vi "Broadcast number of frames and run ID.vi"(8 "error in":errorcluster, 10 "CaptureDetectionLoopDataIn":T1={"Period"=-1, "Reset"=FALSE, "Iteration"=0, "Capture"=path "", "Mode"={"Replay"=enum."None", "Record"=enum."None"}, "Replay Run ID"="", "Frame Number"=0, "Core Module ID"=0, "EventRecorderLaunched"=FALSE, "Frame 0 relative seconds"=0.0} {"Frame 0 relative seconds" format="%_19f"}, 11 "Number of frames":u32) -> (0 "error out":errorcluster)   [LabVIEW 2026, in "Launcher.lvlib"]
doc: "_____\nCreated using DQMH Framework: Event Scripter 7.1.2.1547."
uses:
  Launcher.lvlib
  Capture detection loop data--cluster.ctl
  Mode.ctl
  ReplayMode.ctl
  RecordMode.ctl
  Broadcast number of frames and run ID Argument--cluster.ctl
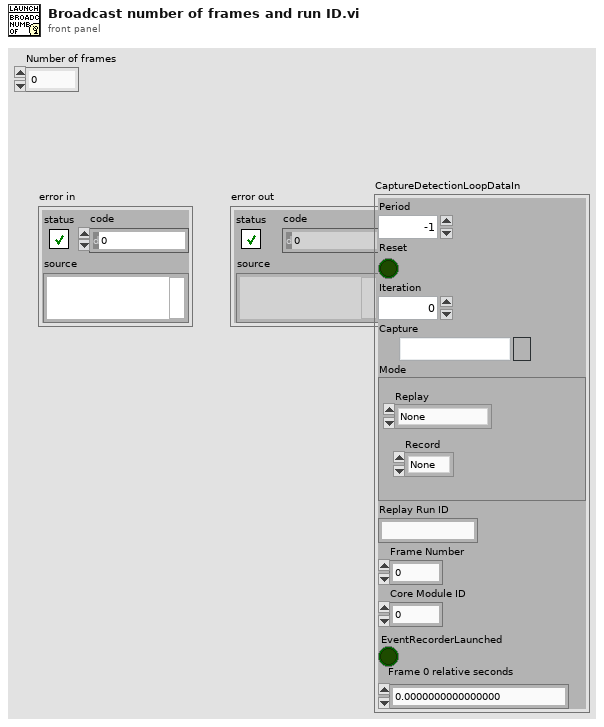
[diagram p1: front panel]
types:
  T1 = typedef "Capture detection loop data--cluster.ctl" = cluster{"Period":i32, "Reset":bool, "Iteration":i32, "Capture":path, "Mode":T2, "Replay Run ID":string, "Frame Number":u32, "Core Module ID":i32, "EventRecorderLaunched":bool, "Frame 0 relative seconds":dbl}
  T2 = typedef "Mode.ctl" = cluster{"Replay":T3, "Record":T4}
  T3 = typedef "ReplayMode.ctl" = enum16{"None", "User Events"}
  T4 = typedef "RecordMode.ctl" = enum16{"None", "User Events", "Benchmarks", "User Events and Benchmarks"}
  T5 = typedef "Launcher.lvlib/Broadcast number of frames and run ID Argument--cluster.ctl" = cluster{"Number of frames":u32, "CaptureDetectionLoopDataIn":T1}
  T6 = typedef "Launcher.lvlib/Broadcast Events--cluster.ctl" = cluster{"Module Did Init":refnum<user-event>, "Status Updated":refnum<user-event>, "Error Reported":refnum<user-event>, "Module Did Stop":refnum<user-event>, "Update Module Execution Status":refnum<user-event>, "Start Capture Detection Loop":refnum<user-event>, "Benchmark Started":refnum<user-event>, "Broadcast number of frames and run ID":refnum<user-event>}
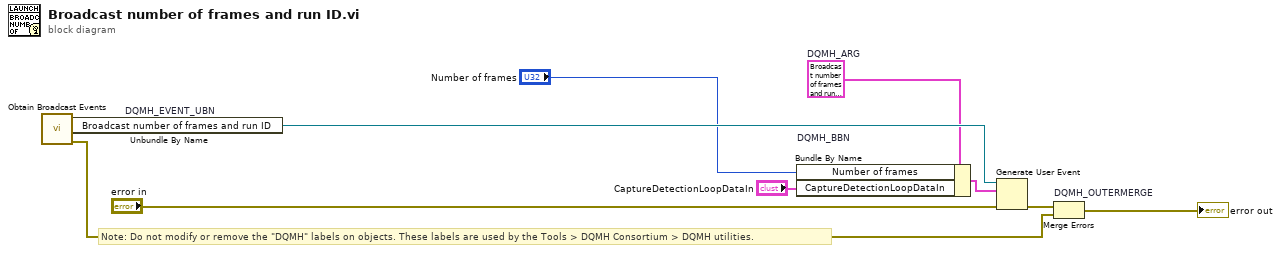
[diagram p0: block diagram]
diagram:
  w5 = T5 {"Number of frames"=0, "CaptureDetectionLoopDataIn"={"Period"=-1, "Reset"=FALSE, "Iteration"=0, "Capture"=path "", "Mode"={"Replay"=enum."None", "Record"=enum."None"}, "Replay Run ID"="", "Frame Number"=0, "Core Module ID"=0, "EventRecorderLaunched"=FALSE, "Frame 0 relative seconds"=0.0}}  # DQMH_ARG
  # "Note: Do not modify or remove the \"DQMH\" labels on objects. These labels are used by the Tools > DQMH Consortium > DQMH utilities."
  n1 = call "Obtain Broadcast Events.vi"() -> ("error out"=w4:errorcluster, "Launcher Broadcast Events"=w3:T6)  [unwired: 10 in]
  n2 = Unbundle By Name "DQMH_EVENT_UBN"(w3) -> ("Broadcast number of frames and run ID"=w7:refnum<user-event>)
  n3 = Bundle By Name "DQMH_BBN"(cluster=w5, "Number of frames"="Number of frames", "CaptureDetectionLoopDataIn"="CaptureDetectionLoopDataIn") -> (w8:T5)
  n4 = Generate User Event(user event=w7, event data cluster=w8, error in="error in") -> (error out=w6:errorcluster)  [unwired: 1 in, 1 out]
  n5 = Merge Errors "DQMH_OUTERMERGE"(w6, w4) -> (→"error out":errorcluster)
